vi "init.vi"(8 "error in":errorcluster, 10 "TBM module configuration in":refnum<class "TBM module configuration.lvclass">, 11 "SQLite runtime in":refnum<class "SQLite runtime.lvclass">) -> (0 "error out":errorcluster, 1 "data allocations":T1, 2 "execution settings":T4, 3 "SQLite runtime out":refnum<class "SQLite runtime.lvclass">)   [LabVIEW 2014, in "SQLite runtime.lvclass"]
doc: "Provides an interface for initializing a module at runtime. While this interface performs no operations, a child should provide an override which may open any necessary references or sessions, allocate necessary memory, and perform any final configuration validataion before providing the full configuration <b>execution data</b> to the calling process."
uses:
  SQLite runtime.lvclass
  <vilib>/NI/Tag Bus Module Framework/module configuration/TBM module configuration.lvclass
  <vilib>/NI/Tag Bus Module Framework/runtime/execution settings.ctl
  <vilib>/NI/Tag Bus Module Framework/channel/data tables.ctl
  <vilib>/NI/Tag Bus/dictionary/data dictionary.lvclass
  <vilib>/NI/Tag Bus/dictionary table pair.ctl
  <vilib>/NI/Tag Bus/table/data table.ctl
  configuration/SQLite configuration.lvclass
  SQLite runtime.lvclass/SQLite runtime.ctl
  <vilib>/drjdpowell/SQLite Library/SQL Connection/Open (string).vi
  <vilib>/drjdpowell/SQLite Library/SQL Connection/Execute SQL (No results).vi
  <vilib>/drjdpowell/SQLite Library/SQL Connection/Connection.lvclass
  <vilib>/NI/Tag Bus Module Framework/channel/TBM channel.lvclass
  <vilib>/NI/Tag Bus Module Framework/runtime/TBM module execution interface.lvclass
  <vilib>/drjdpowell/SQLite Library/SQLite.lvlib
  <vilib>/NI/Tag Bus/tag bus.lvlib
  <vilib>/NI/Tag Bus/table/data table.lvlib
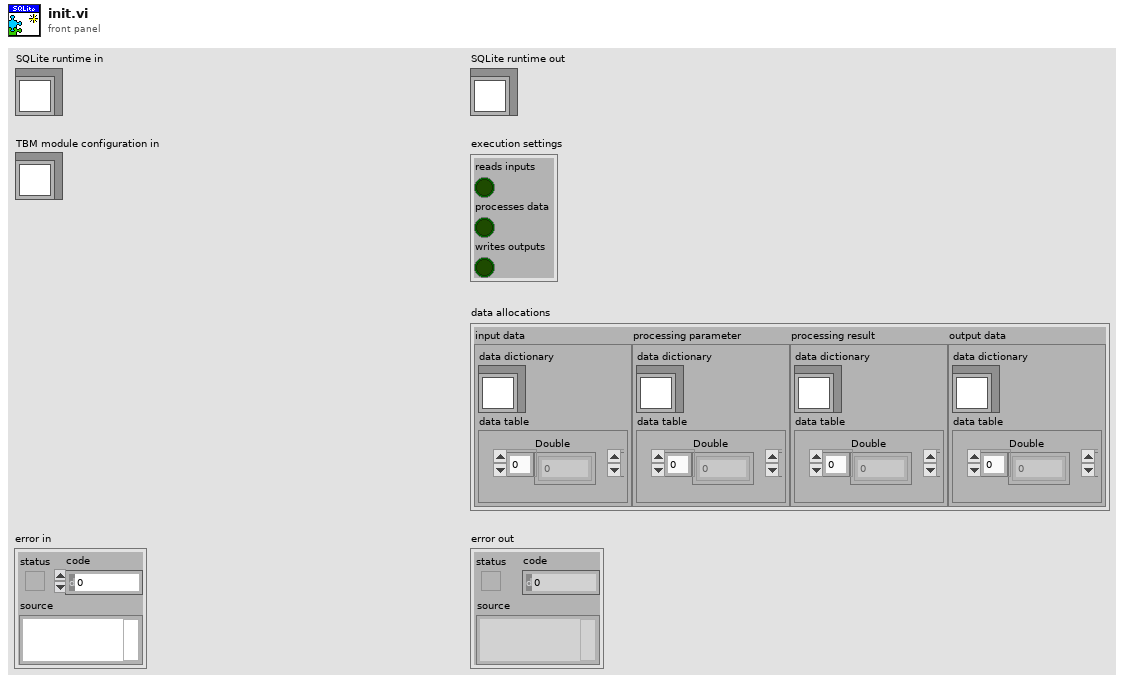
[diagram p1: front panel]
types:
  T1 = typedef "TBM channel.lvclass/data tables.ctl" = cluster{"input data":T2, "processing parameter":T2, "processing result":T2, "output data":T2}
  T2 = typedef "tag bus.lvlib/dictionary table pair.ctl" = cluster{"data dictionary":refnum<class "data dictionary.lvclass">, "data table":T3}
  T3 = typedef "tag bus.lvlib/data table.lvlib/data table.ctl" = cluster{"Double":dbl[], "Single":sgl[], "I64":i64[], "I32":i32[], "I16":i16[], "I8":i8[], "U64":u64[], "U32":u32[], "U16":u16[], "U8":u8[], "Boolean":bool[], "String":string[], "Array of Double":cluster{"DBL Array":dbl[]}[], "Array of Single":cluster{"SGL Array":sgl[]}[], "Array of I64":cluster{"I64 Array":i64[]}[], "Array of I32":cluster{"I32 Array":i32[]}[], "Array of I16":cluster{"I16 Array":i16[]}[], "Array of I8":cluster{"I8 Array":i8[]}[], "Array of U64":cluster{"U64 Array":u64[]}[], "Array of U32":cluster{"U32 Array":u32[]}[], "Array of U16":cluster{"U16 Array":u16[]}[], "Array of U8":cluster{"U8 Array":u8[]}[], "Array of Boolean":cluster{"Boolean Array":bool[]}[], "Array of String":cluster{"String Array":string[]}[]}
  T4 = typedef "TBM module execution interface.lvclass/execution settings.ctl" = cluster{"reads inputs":bool, "processes data":bool, "writes outputs":bool}
  T5 = typedef "SQLite runtime.lvclass/data map.ctl" = cluster{"DCAF Type":T6, "Index":i32, "SQLite Type":T7, "db key":string}
  T6 = typedef "tag bus.lvlib/tag descriptor.lvclass/Data Type.ctl" = enum16{"Double", "Single", "I64", "I32", "I16", "I8", "U64", "U32", "U16", "U8", "Boolean", "String", "Array of Double", "Array of Single", "Array of I64", "Array of I32", "Array of I16", "Array of I8", "Array of U64", "Array of U32", "Array of U16", "Array of U8", "Array of Boolean", "Array of String"}
  T7 = typedef "SQLite runtime.lvclass/sqlite type.ctl" = enum16{"DBL", "I64", "String"}
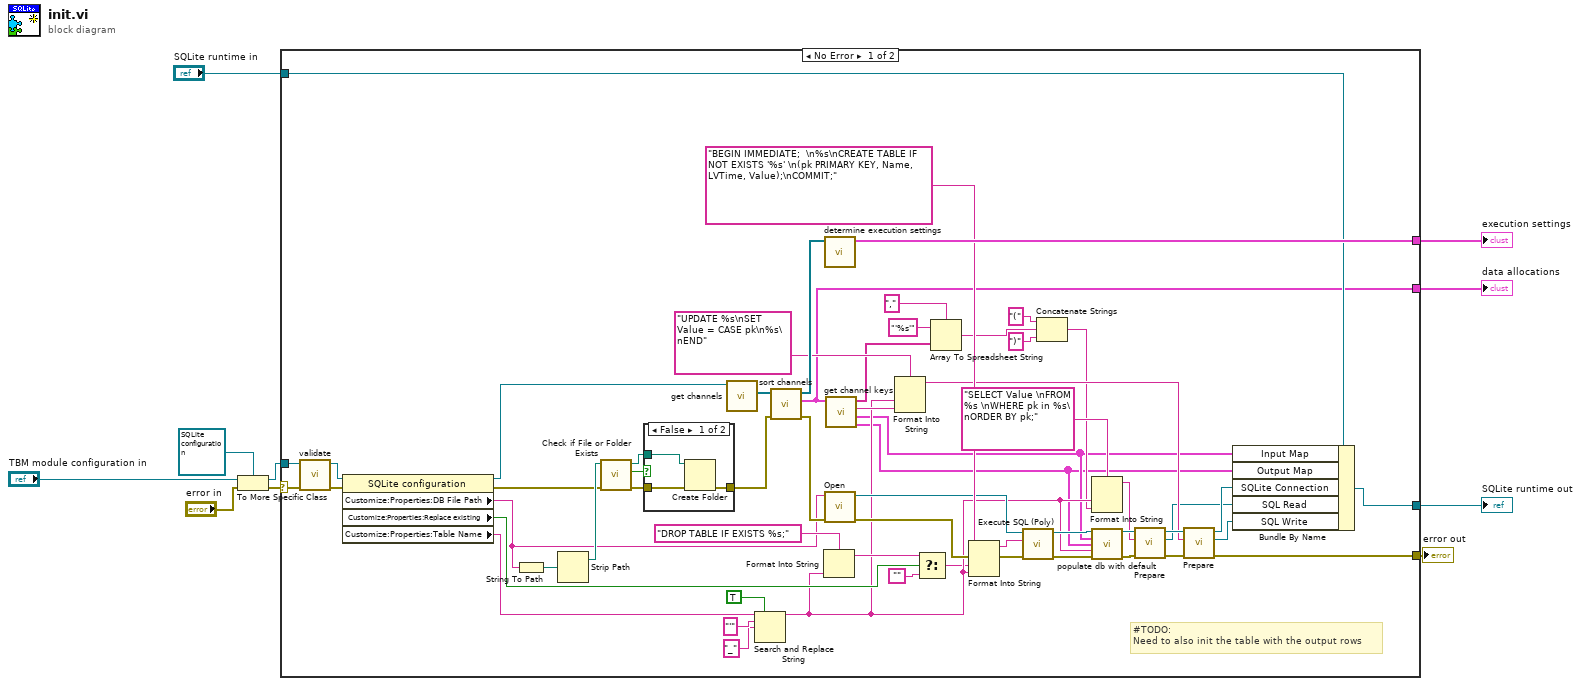
[diagram p0: block diagram]
diagram:
  n1 = To More Specific Class(target class=refnum<class "SQLite configuration.lvclass"> refnum ("Synchronous module configuration"), reference="TBM module configuration in", error in="error in") -> (specific class reference=w9:refnum<class "SQLite configuration.lvclass">, error out=w10:errorcluster)
  n2 = case shown="No Error" w10 {
    selector: w10 -> [w67 w74]
    tunnel: w9 -> [w66 _]
    tunnel: "SQLite runtime in" -> [w61 w75]
    tunnel: [w60 w75] -> w4
    tunnel: [w58 w74] -> w3
    tunnel: [w39 _] -> w1
    tunnel: [w69 _] -> w2
    frame No Error {
      # "#TODO:\nNeed to also init the table with the output rows"
      n3 = call-dynamic "validate.vi"("error in"=w67, "SQLite configuration in"=w66) -> ("error out"=w63:errorcluster, "SQLite configuration out"=w64:refnum<class "SQLite configuration.lvclass">)  [unwired: 8 in]
      n4 = property class="SQLite configuration"(reference=w64, error in=w63) -> (reference out=w62:refnum<class "SQLite configuration.lvclass">, error out=w15:errorcluster, "Customize:Properties:DB File Path"=w16:string, "Customize:Properties:Replace existing"=w48:bool, "Customize:Properties:Table Name"=w47:string)
      n5 = String To Path(string=w16) -> (path=w17:path)
      n6 = Strip Path(path=w17) -> (stripped path=w21:path)  [unwired: 1 out]
      n7 = call <vilib>:"Check if File or Folder Exists.vi"("error in (no error)"=w15, "path"=w21) -> ("error out"=w18:errorcluster, "file or folder exists?"=w20:bool, "dup path"=w19:path)  [unwired: 7 in]
      n8 = case shown="False" w20 {
        tunnel: w19 -> [w72 _]
        tunnel: w18 -> [w71 w73]
        tunnel: [w70 w73] -> w14
        frame False {
          n9 = Create Folder(path (use dialog)=w72, error in=w71) -> (error out=w70:errorcluster)  [unwired: 1 in, 2 out]
        }
        frame True {
        }
      }
      n10 = call-dynamic "get channels.vi"("SQLite configuration in"=w62) -> ("channels"=w65:refnum<class "TBM channel.lvclass">[])  [unwired: 9 in, 1 out]
      n11 = Search and Replace String(replace all?=TRUE ("replace all? (F)"), input string=w47, search string="'", replace string="_" ("replace string (\"\")")) -> (result string=w24:string)  [unwired: 4 in, 3 out]
      n12 = call <vilib>:"sort channels.vi"("error in"=w14, "channels in"=w65) -> ("error out"=w59:errorcluster, "data allocations"=w39:T1, "channels out"=w68:refnum<class "TBM channel.lvclass">[])  [unwired: 7 in]
      n13 = Format Into String(format string="DROP TABLE IF EXISTS %s;" ("SQL"), w24) -> (resulting string=w43:string)  [unwired: 2 in, 1 out]
      n14 = call <vilib>:"determine execution settings.vi"("channels"=w68) -> ("execution settings"=w69:T4)  [unwired: 10 in]
      n15 = call-poly <vilib>:"Open.vi"("error in (no error)"=w59, "db file"=w16) -> ("error out"=w50:errorcluster, "SQLite Connection out"=w51:refnum<class "Connection.lvclass">)  [unwired: 8 in]
      n16 = call "get channel keys.vi"("data allocations"=w39) -> ("Output Map"=w11:T5[], "Input Map"=w12:T5[], "output subquery"=w36:string, "input pk list"=w29:string[])  [unwired: 7 in]
      n17 = Format Into String(format string="UPDATE %s\nSET Value = CASE pk\n%s\nEND" ("SQL"), w24, w36) -> (resulting string=w40:string)  [unwired: 2 in, 1 out]
      n18 = Select(t=w43, s=w48, f="") -> (s? t:f=w13:string)
      n19 = Array To Spreadsheet String(delimiter (Tab)=",", array=w29, 3:"'%s'" ("format string")) -> (spreadsheet string=w28:string)
      n20 = Format Into String(format string="BEGIN IMMEDIATE;  \n%s\nCREATE TABLE IF NOT EXISTS '%s' \n(pk PRIMARY KEY, Name, LVTime, Value);\nCOMMIT;" ("SQL"), error in=w50, w13, w24) -> (resulting string=w52:string, error out=w49:errorcluster)  [unwired: 1 in]
      n21 = call-poly <vilib>:"Execute SQL (Poly).vi"("error in (no error)"=w49, "SQL"=w52, "SQLite Connection in"=w51) -> ("error out"=w33:errorcluster, "SQLite Connection out"=w35:refnum<class "Connection.lvclass">)  [unwired: 7 in]
      n22 = Concatenate Strings("(" ("string"), w28, ")" ("string")) -> (w22:string)
      n23 = Format Into String(format string="SELECT Value \nFROM %s \nWHERE pk in %s\nORDER BY pk;" ("SQL"), w24, w22) -> (resulting string=w23:string)  [unwired: 2 in, 1 out]
      n24 = call "populate db with default.vi"("SQLite Connection in"=w35, "Input Map"=w12, "Output Map"=w11, "table name"=w24, "error in"=w33) -> ("SQLite Connection out"=w34:refnum<class "Connection.lvclass">, "error out"=w32:errorcluster)  [unwired: 9 in]
      n25 = call <vilib>:"Prepare.vi"("error in (no error)"=w32, "SQL"=w23, "SQLite Connection in"=w34) -> ("error out"=w37:errorcluster, "SQL Statement out"=w38:refnum<class "SQL Statement.lvclass">, "SQLite Connection out"=w55:refnum<class "Connection.lvclass">)  [unwired: 4 in, 2 out]
      n26 = call <vilib>:"Prepare.vi"("error in (no error)"=w37, "SQL"=w40, "SQLite Connection in"=w55) -> ("error out"=w58:errorcluster, "SQL Statement out"=w57:refnum<class "SQL Statement.lvclass">, "SQLite Connection out"=w56:refnum<class "Connection.lvclass">)  [unwired: 4 in, 2 out]
      n27 = Bundle By Name(cluster=w61, "Input Map"=w12, "Output Map"=w11, "SQLite Connection"=w56, "SQL Read"=w38, "SQL Write"=w57) -> (w60:refnum<class "SQLite runtime.lvclass">)
    }
    frame Error {
    }
  }
  "error out" <- w3
  "SQLite runtime out" <- w4
  "execution settings" <- w2
  "data allocations" <- w1
